vi "OwnInterface20261013_Info.vi"() -> ()   [LabVIEW 2024]
panel:
  out "error out":errorcluster caption="错误输出"
  out "Count":i32
  out "Is Interface":bool
  in  "Class Path":path
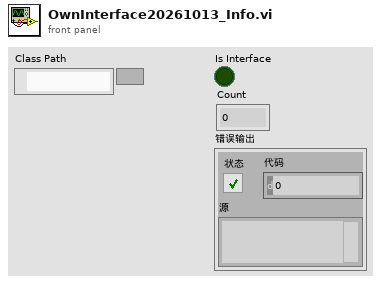
[diagram p1: front panel]
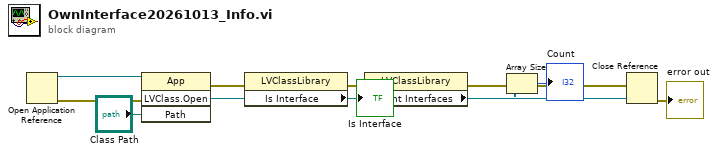
[diagram p0: block diagram]
diagram:
  n1 = Open Application Reference() -> (0:w9:errorcluster, 3:w11:refnum<vi>)  [unwired: 4 in]
  n2 = invoke class="App" method="LVClass.Open"(reference=w11, error in=w9, "Path"="Class Path") -> (error out=w7:errorcluster, "LVClass.Open"=w8:refnum<vi>)  [unwired: 1 in, 2 out]
  n3 = property class="LVClassLibrary"(reference=w8, error in=w7) -> (error out=w5:errorcluster, "Is Interface"=→"Is Interface":bool)  [unwired: 1 out]
  n4 = property class="LVClassLibrary"(reference=w8, error in=w5) -> (error out=w2:errorcluster, "Parent Interfaces"=w4:refnum<vi>[])  [unwired: 1 out]
  n5 = Array Size(array=w4) -> (size(s)=→"Count":i32)
  n6 = Close Reference(reference=w8, error in (no error)=w2) -> (error out=→"error out":errorcluster)
